vi "Cleanup Client If Error.vi"(8 "error in":errorcluster, 10 "client name":string, 11 "project ref in":refnum<vi>) -> (0 "error out":errorcluster, 3 "project ref out":refnum<vi>)   [LabVIEW 2021, in "NI Measurement V2 Client Generator Runtime.lvlib"]
uses:
  NI Measurement V2 Client Generator Runtime.lvlib
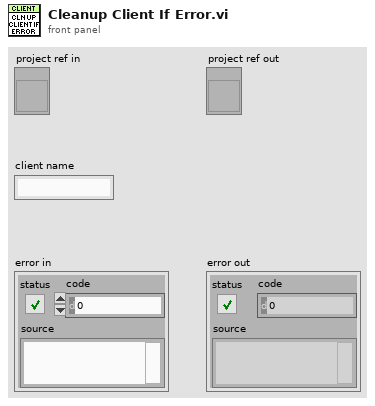
[diagram p1: front panel]
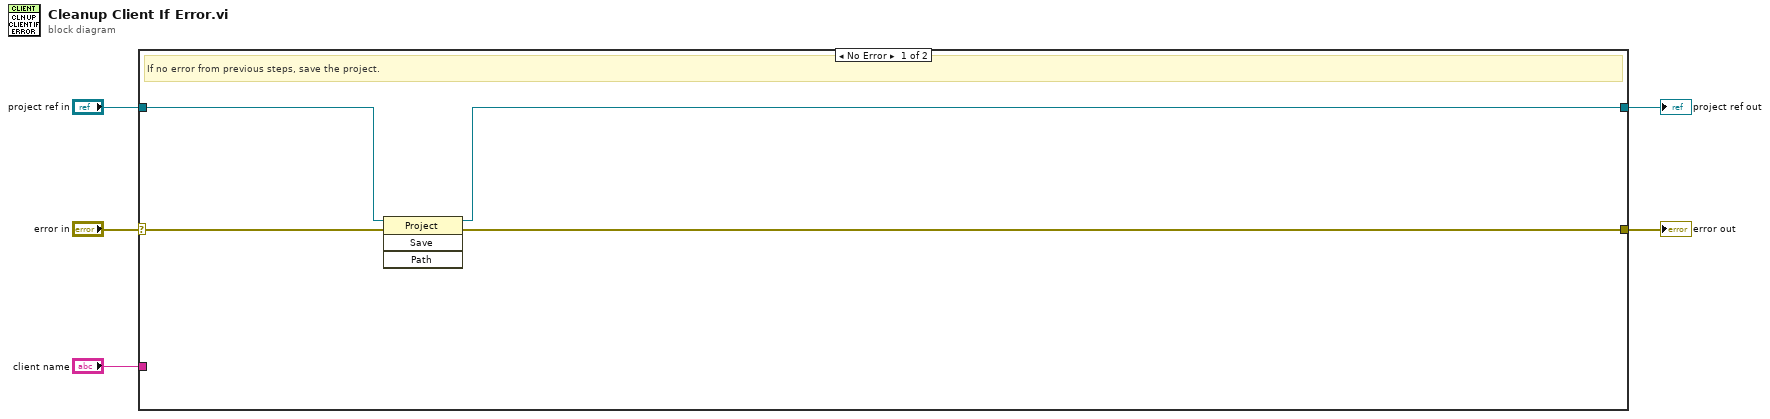
[diagram p0: block diagram]
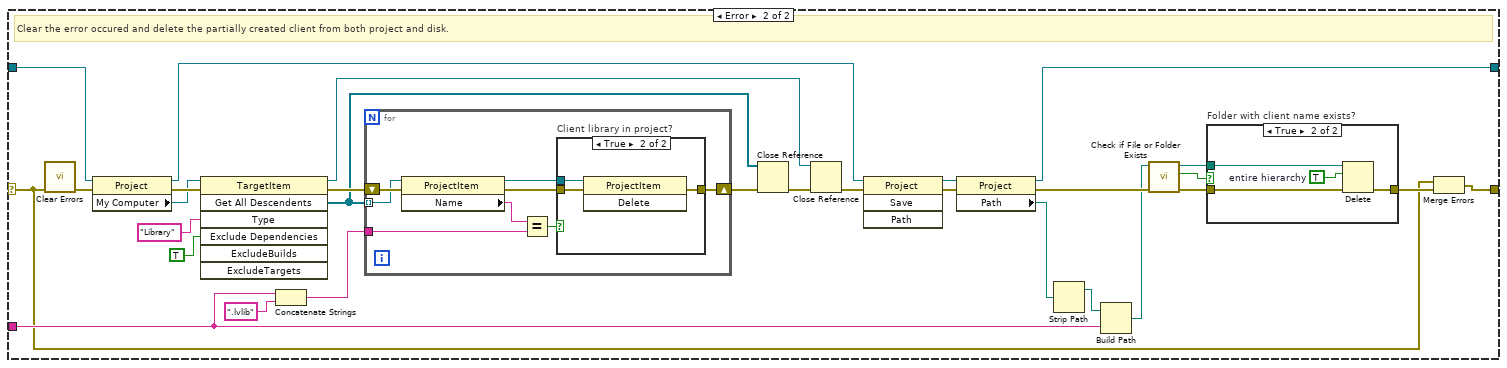
[diagram p2: hidden frame]
diagram:
  n1 = case shown="No Error" "error in" {
    selector: "error in" -> [w9 w12]
    tunnel: "project ref in" -> [w8 w38]
    tunnel: [w7 w31] -> w4
    tunnel: "client name" -> [_ w16]
    tunnel: [w6 w17] -> w2
    frame No Error {
      # "If no error from previous steps, save the project."
      n2 = invoke class="Project" method="Save"(reference=w8, error in=w9) -> (reference out=w7:refnum<vi>, error out=w6:errorcluster)  [unwired: 2 in, 2 out]
    }
    frame Error {
      # "Clear the error occured and delete the partially created client from both project and disk."
      n3 = call <vilib>:"Clear Errors.vi"("error in (no error)"=w12) -> ("error out"=w11:errorcluster)  [unwired: 5 in, 1 out]
      n4 = property class="Project"(reference=w38, error in=w11) -> (reference out=w24:refnum<vi>, error out=w14:errorcluster, "My Computer"=w13:refnum<vi>)
      n5 = invoke class="TargetItem" method="Get All Descendents"(reference=w13, error in=w14, "Type"="Library", "Exclude Dependencies"=TRUE ("ExcludeDependencies")) -> (reference out=w33:refnum<vi>, error out=w15:errorcluster, "All Descendents"=w10:refnum<vi>[])  [unwired: 3 in, 4 out]
      n6 = Concatenate Strings(w16, ".lvlib" ("string")) -> (w21:string)
      n7 = for {
        tunnel: w10 -> [w39] mode=indexing
        tunnel: w21 -> [w45]
        shift-right: [w41] -> w35
        shift-left: w15 -> [w40]
        n8 = property class="ProjectItem"(reference=w39, error in=w40) -> (reference out=w44:refnum<vi>, error out=w42:errorcluster, "Name"=w46:string)
        n9 = Equal?(x=w46, y=w45) -> (x = y?=w43:bool)
        n10 = case "Client library in project?" shown="True" w43 {
          tunnel: w44 -> [_ w50]
          tunnel: w42 -> [w47 w49]
          tunnel: [w47 w48] -> w41
          frame False {
          }
          frame True {
            n11 = invoke class="ProjectItem" method="Delete"(reference=w50, error in=w49) -> (error out=w48:errorcluster)  [unwired: 1 in, 2 out]
          }
        }
      }
      n12 = Close Reference(reference=w10, error in (no error)=w35) -> (error out=w19:errorcluster)
      n13 = Close Reference(reference=w33, error in (no error)=w19) -> (error out=w34:errorcluster)
      n14 = invoke class="Project" method="Save"(reference=w24, error in=w34) -> (reference out=w23:refnum<vi>, error out=w25:errorcluster)  [unwired: 2 in, 2 out]
      n15 = property class="Project"(reference=w23, error in=w25) -> (reference out=w31:refnum<vi>, error out=w32:errorcluster, "Path"=w30:path)
      n16 = Strip Path(path=w30) -> (stripped path=w29:path)  [unwired: 1 out]
      n17 = Build Path(base path=w29, name or relative path=w16) -> (appended path=w28:path)
      n18 = call <vilib>:"Check if File or Folder Exists.vi"("error in (no error)"=w32, "path"=w28) -> ("error out"=w27:errorcluster, "file or folder exists?"=w20:bool, "dup path"=w26:path)  [unwired: 7 in]
      n19 = case "Folder with client name exists?" shown="True" w20 {
        tunnel: w27 -> [w51 w55]
        tunnel: [w51 w54] -> w18
        tunnel: w26 -> [_ w53]
        frame False {
        }
        frame True {
          w52 = TRUE  # entire hierarchy
          n20 = Delete(path (use dialog)=w53, entire hierarchy (F)=w52, error in=w55) -> (error out=w54:errorcluster)  [unwired: 2 in, 2 out]
        }
      }
      n21 = Merge Errors(w12, w18) -> (w17:errorcluster)
    }
  }
  "project ref out" <- w4
  "error out" <- w2
